vi "Item_Init.vi"(11 "Object":T1) -> ()   [LabVIEW 2020, in "Project Provider.lvlib"]
uses:
  Project Provider.lvlib
  <resource>/Framework/Providers/API/mxLvUpdateUI.ctl
  <resource>/Framework/Providers/API/mxLvOverlayState.ctl
  LUnit Test Case.lvclass
  <resource>/Framework/Providers/API/ItemRef.ctl
panel:
  out "error out":errorcluster
  in  "error in":errorcluster
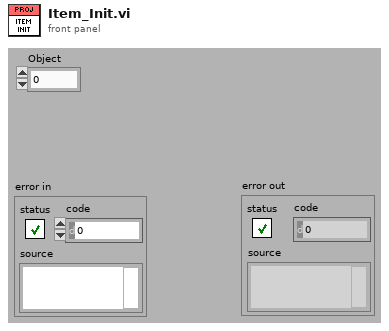
[diagram p1: front panel]
types:
  T1 = typedef "ItemRef.ctl" = u64
  T2 = typedef "mxLvUpdateUI.ctl" = cluster{"Action":u32, "Optional param 1":string, "Optional param 2":i32, "Optional param 3":string}
  T3 = typedef "mxLvOverlayState.ctl" = cluster{"Overlay Alias":string, "Active":bool}
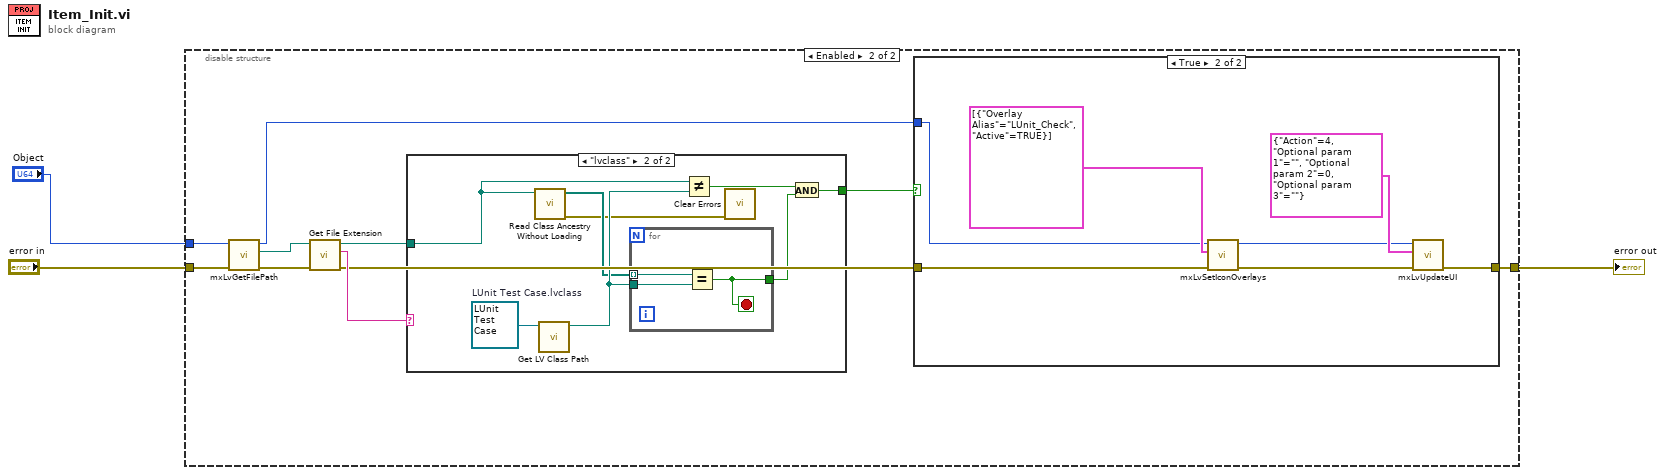
[diagram p0: block diagram]
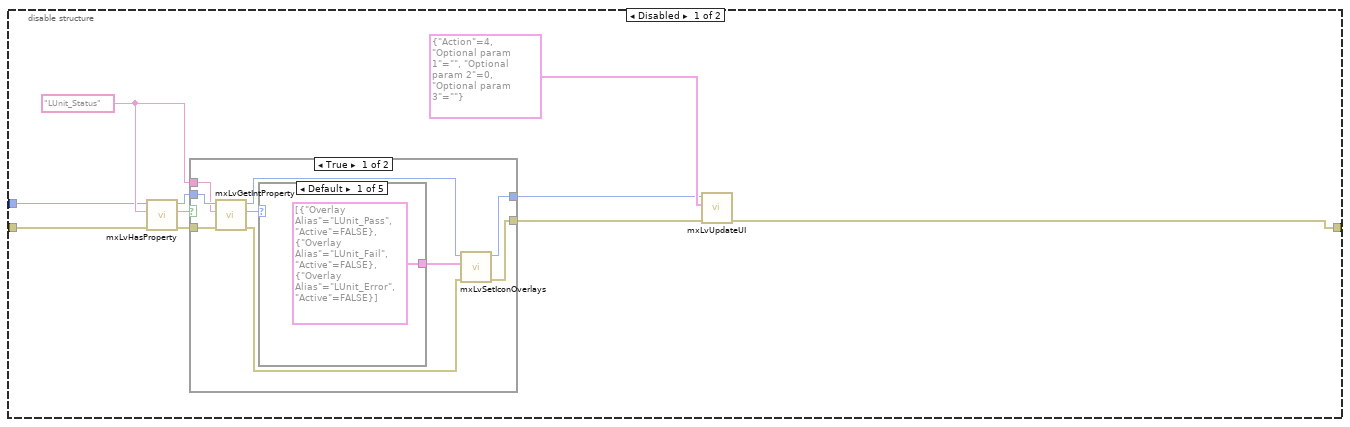
[diagram p2: hidden frame]
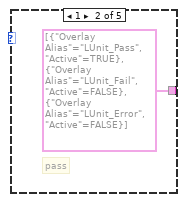
[diagram p3: hidden frame]
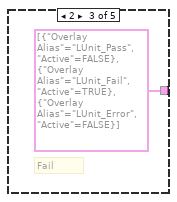
[diagram p4: hidden frame]
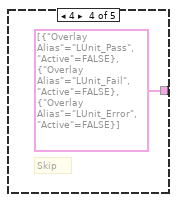
[diagram p5: hidden frame]
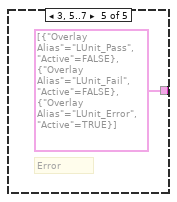
[diagram p6: hidden frame]
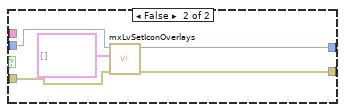
[diagram p7: hidden frame]
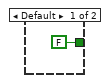
[diagram p9: hidden frame]
diagram:
  n1 = disable-structure shown="Enabled" {
    disable-tunnel: "error in" -> [w13 w41]
    disable-tunnel: [w12 w35] -> w1
    disable-tunnel: "Object" -> [w4 w42]
    frame Disabled {
      w7 = "LUnit_Status" ("Tag")
      n2 = call <resource>:"mxLvHasProperty.vi"("error in"=w13, "Tag"=w7, "Item"=w4) -> ("error out"=w6:errorcluster, "HasProperty"=w11:bool, "Item"=w5:T1)  [unwired: 6 in]
      n3 = case shown="True" w11 {
        tunnel: w5 -> [w22 w30]
        tunnel: w6 -> [w21 w29]
        tunnel: w7 -> [w20 _]
        tunnel: [w19 w32] -> w8
        tunnel: [w18 w31] -> w9
        frame True {
          n4 = call <resource>:"mxLvGetIntProperty.vi"("error in"=w21, "Tag"=w20, "Item"=w22) -> ("error out"=w15:errorcluster, "Value"=w14:i32, "Item"=w16:T1)  [unwired: 6 in]
          n5 = case shown="Default" w14 {
            tunnel: [T3[] [{"Overlay Alias"="LUnit_Pass", "Active"=FALSE}, {"Overlay Alias"="LUnit_Fail", "Active"=FALSE}, {"Overlay Alias"="LUnit_Error", "Active"=FALSE}] ("Array") T3[] [{"Overlay Alias"="LUnit_Pass", "Active"=TRUE}, {"Overlay Alias"="LUnit_Fail", "Active"=FALSE}, {"Overlay Alias"="LUnit_Error", "Active"=FALSE}] ("Array") T3[] [{"Overlay Alias"="LUnit_Pass", "Active"=FALSE}, {"Overlay Alias"="LUnit_Fail", "Active"=TRUE}, {"Overlay Alias"="LUnit_Error", "Active"=FALSE}] ("Array") T3[] [{"Overlay Alias"="LUnit_Pass", "Active"=FALSE}, {"Overlay Alias"="LUnit_Fail", "Active"=FALSE}, {"Overlay Alias"="LUnit_Error", "Active"=FALSE}] ("Array") T3[] [{"Overlay Alias"="LUnit_Pass", "Active"=FALSE}, {"Overlay Alias"="LUnit_Fail", "Active"=FALSE}, {"Overlay Alias"="LUnit_Error", "Active"=TRUE}] ("Array")] -> w17
            frame Default {
            }
            frame 1 {
              # "pass"
            }
            frame 2 {
              # "Fail"
            }
            frame 4 {
              # "Skip"
            }
            frame 3, 5..7 {
              # "Error"
            }
          }
          n6 = call <resource>:"mxLvSetIconOverlays.vi"("error in"=w15, "Overlay States"=w17, "Item"=w16) -> ("error out"=w19:errorcluster, "Item"=w18:T1)  [unwired: 7 in]
        }
        frame False {
          n7 = call <resource>:"mxLvSetIconOverlays.vi"("error in"=w29, "Overlay States"=T3[] [], "Item"=w30) -> ("error out"=w32:errorcluster, "Item"=w31:T1)  [unwired: 7 in]
        }
      }
      n8 = call <resource>:"mxLvUpdateUI.vi"("error in"=w8, "Update UI Settings"=T2 {"Action"=4, "Optional param 1"="", "Optional param 2"=0, "Optional param 3"=""}, "Item"=w9) -> ("error out"=w12:errorcluster)  [unwired: 7 in, 1 out]
    }
    frame Enabled {
      n9 = call <resource>:"mxLvGetFilePath.vi"("error in"=w41, "Item"=w42) -> ("error out"=w40:errorcluster, "File Path"=w39:path, "Item"=w34:T1)  [unwired: 7 in]
      n10 = call <vilib>:"Get File Extension.vi"("error in (no error)"=w40, "file"=w39) -> ("error out"=w36:errorcluster, "lowercase file extension"=w37:string, "dup file"=w38:path)  [unwired: 5 in, 2 out]
      n11 = case shown="\"lvclass\"" w37 {
        tunnel: w38 -> [_ w53]
        tunnel: [FALSE w52] -> w33
        frame Default {
        }
        frame "lvclass" {
          w59 = refnum<class "LUnit Test Case.lvclass"> refnum  # LUnit Test Case.lvclass
          n12 = call <vilib>:"Read Class Ancestry Without Loading.vi"("LabVIEW Class Path"=w53) -> ("error out"=w55:errorcluster, "Class Ancestry"=w57:path[])  [unwired: 9 in]
          n13 = call <vilib>:"Get LV Class Path.vi"("object"=w59) -> ("class path"=w58:path)  [unwired: 9 in, 1 out]
          n14 = for {
            tunnel: w57 -> [w62] mode=indexing
            tunnel: w58 -> [w61]
            tunnel: [w60] -> w56
            stop <- w60 stop-if-true
            n15 = Equal?(x=w62, y=w61) -> (x = y?=w60:bool)
          }
          n16 = Not Equal?(x=w53, y=w58) -> (x != y?=w54:bool)
          n17 = call <vilib>:"Clear Errors.vi"("error in (no error)"=w55) -> ()  [unwired: 5 in, 2 out]
          n18 = And(x=w54, y=w56) -> (x .and. y?=w52:bool)
        }
      }
      n19 = case shown="True" w33 {
        tunnel: w36 -> [w43 w48]
        tunnel: [w43 w46] -> w35
        tunnel: w34 -> [_ w45]
        frame False {
        }
        frame True {
          n20 = call <resource>:"mxLvSetIconOverlays.vi"("error in"=w48, "Overlay States"=T3[] [{"Overlay Alias"="LUnit_Check", "Active"=TRUE}] ("Array"), "Item"=w45) -> ("error out"=w47:errorcluster, "Item"=w44:T1)  [unwired: 7 in]
          n21 = call <resource>:"mxLvUpdateUI.vi"("error in"=w47, "Update UI Settings"=T2 {"Action"=4, "Optional param 1"="", "Optional param 2"=0, "Optional param 3"=""}, "Item"=w44) -> ("error out"=w46:errorcluster)  [unwired: 7 in, 1 out]
        }
      }
    }
  }
  "error out" <- w1
